vi "Initialise.vi"(8 "error in (no error)":errorcluster, 11 "Viewmodel":refnum<class "Viewmodel.lvclass">) -> (0 "error out":errorcluster, 3 "View out":refnum<class "View.lvclass">)   [LabVIEW 2024, in "View.lvclass"]
uses:
  View.lvclass
  Viewmodel/Viewmodel.lvclass
  View.lvclass/View.ctl
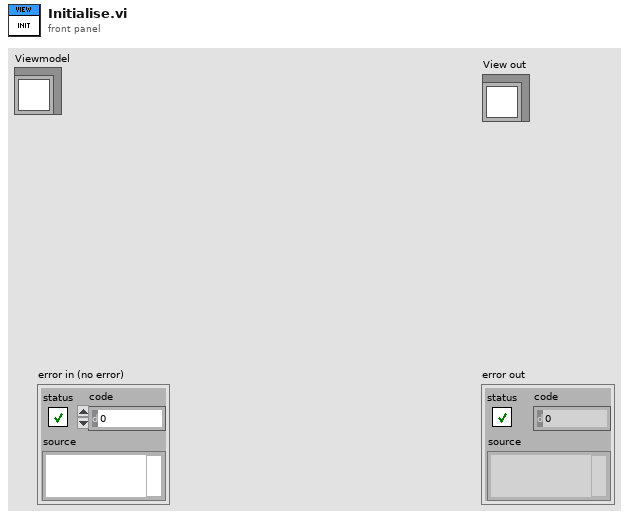
[diagram p1: front panel]
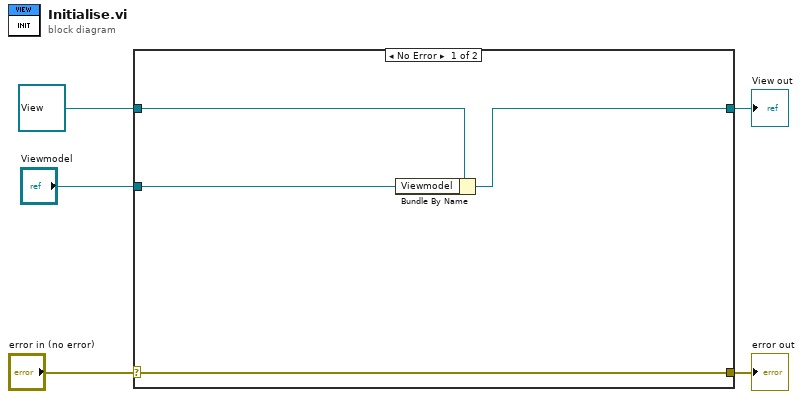
[diagram p0: block diagram]
diagram:
  n1 = case shown="No Error" "error in (no error)" {
    selector: "error in (no error)" -> [w9 w11]
    tunnel: [w9 w11] -> w4
    tunnel: [w6 w10] -> w2
    tunnel: refnum<class "View.lvclass"> refnum ("View in") -> [w8 w10]
    tunnel: "Viewmodel" -> [w7 _]
    frame No Error {
      n2 = Bundle By Name(cluster=w8, "Viewmodel"=w7) -> (w6:refnum<class "View.lvclass">)
    }
    frame Error {
    }
  }
  "error out" <- w4
  "View out" <- w2
